vi "Upload_test_VI.vi"(8 "error in":errorcluster, 11 "SHz_selection":enum16{"10k", "100k"}(ring)) -> (0 "error out":errorcluster, 2 "selected F_array_Link":path[](array[path]), 3 "selected folder_List":string[](array[string]))   [LabVIEW 2018]
panel:
  in  "Add All Sample":bool
  in  "Add All":bool
  out "FOL#":i32
  out "x-1":u32
  out "SIDE":i32
  in  "Scrollbar V":i32(c297)
  out "Selected EX#":i32
  out "element":string
  in  "END":bool
  in  "All_Clear":bool
  in  "EX_IDX":i32
  out "Height":u32
  out "Top":i32
  out "Vertical":i32
  in  "selection":u16(ring) items=["backup (Rackstation)", "BR", "cadet", "COVID19", "Gynecologic Cancer", "HU", "KATO", "KATO2", "KATO3", "komoto", "Konno", "Kumamoto", "Kumamoto_N", "Lee", "Lee2", "Lee3", "LG_EX", "Lipid", "Numata_CHR", "Numata_MF", "Numata_N", "oligopeptide", "Pan_Cancer_N2", "Phi174", "Ryu", "Smoking"]
  out "1folder names":string[](array[string])
  out "Folder_List":string[](array[string])
  out "F_array_Link":path[](array[path])
  out "1st":path[](array[path])
  out "2nd":path[](array[path])
  out "logical OR 2":bool
  out "logical OR":bool
  out "foldername":string[](array[string])
  out "path":path
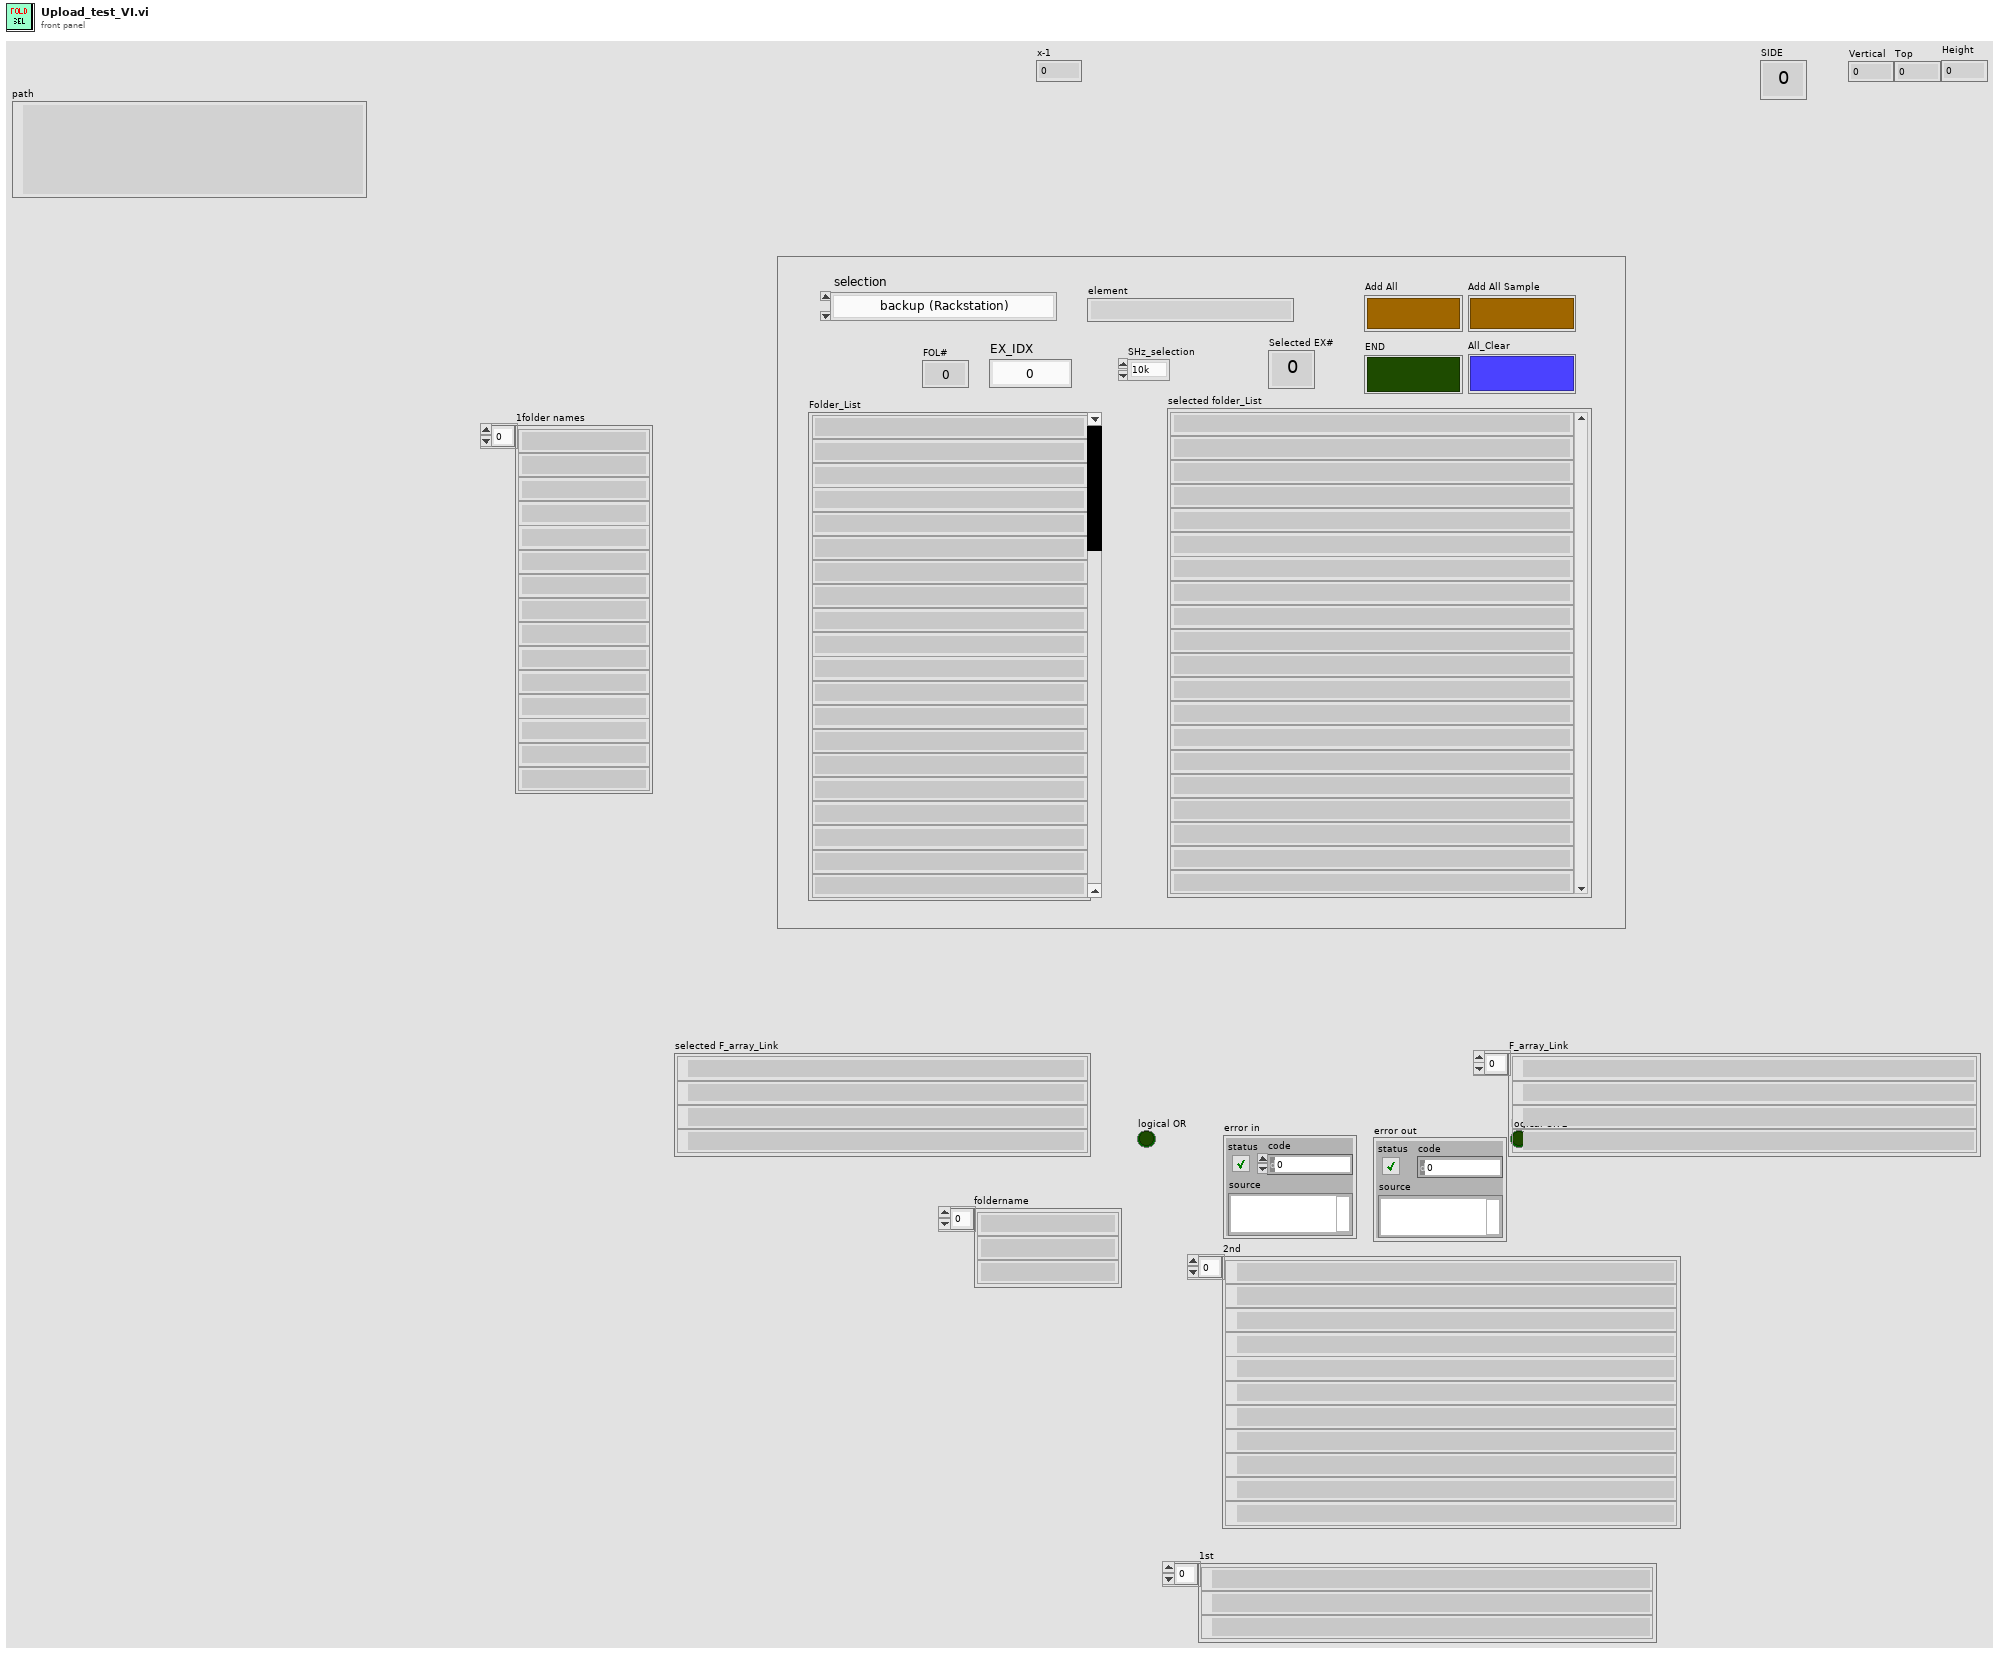
[diagram p1: front panel]
types:
  T1 = typedef "LVPoint32TypeDef.ctl" = cluster{"Horizontal":i32, "Vertical":i32}
  T2 = typedef "LVPositionTypeDef.ctl" = cluster{"Left":i32, "Top":i32}
  T3 = typedef "LVBoundsTypeDef.ctl" = cluster{"Width":u32, "Height":u32}
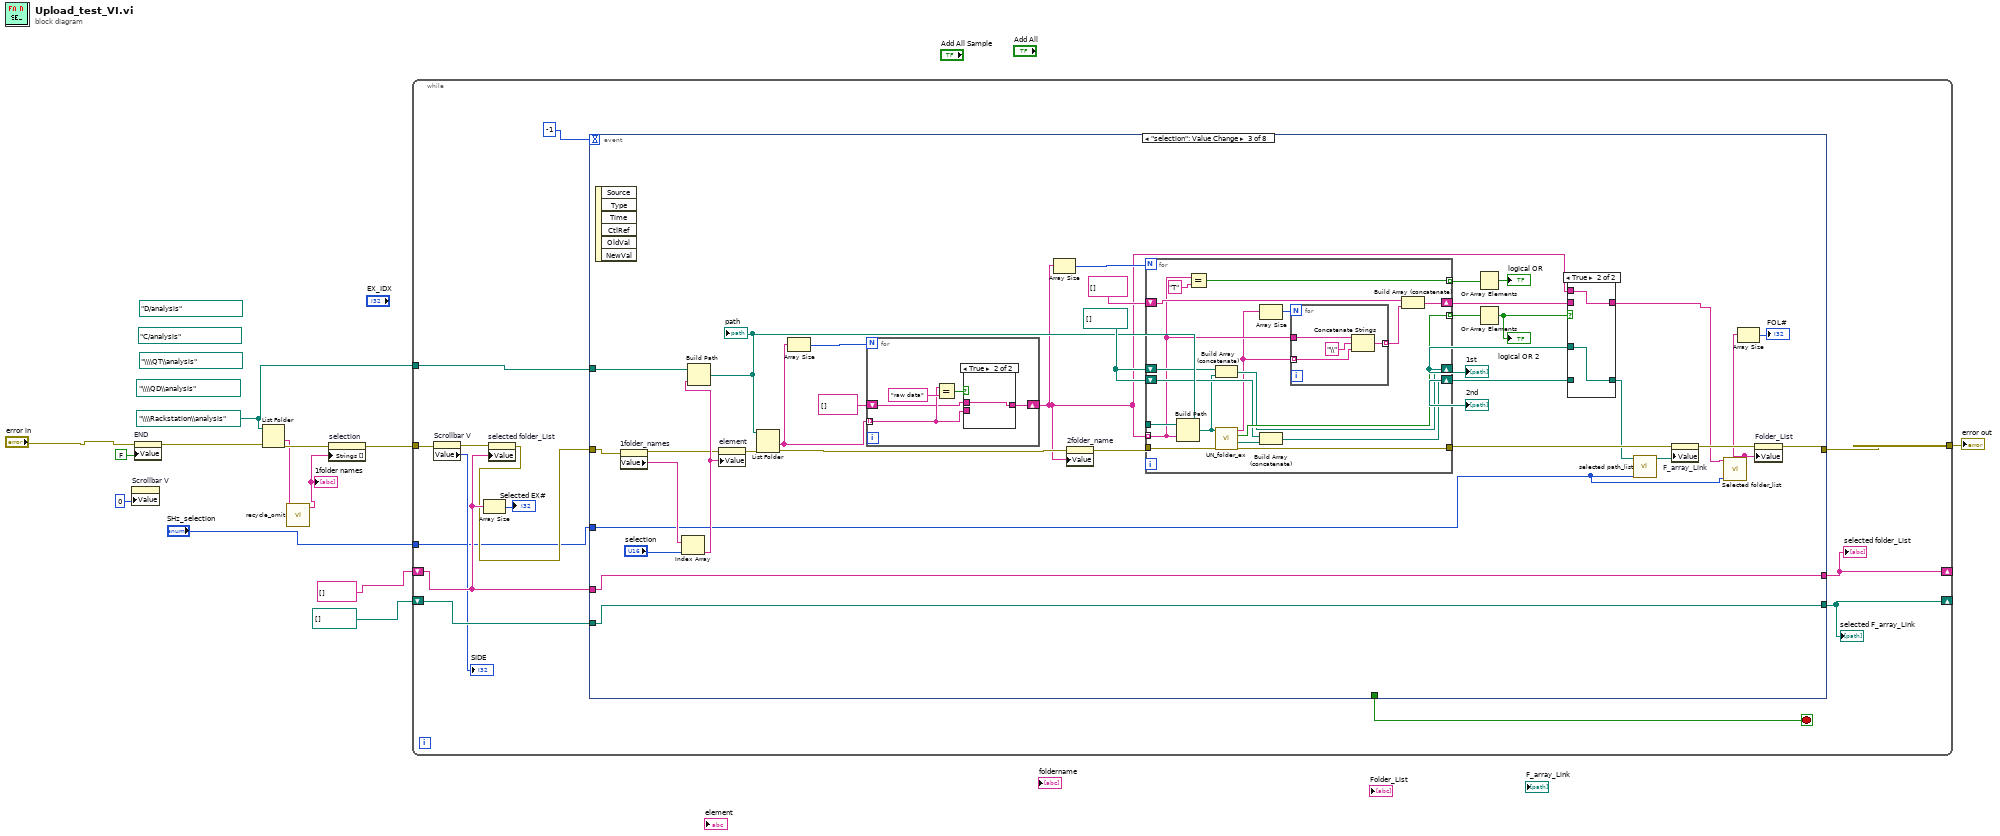
[diagram p0: block diagram]
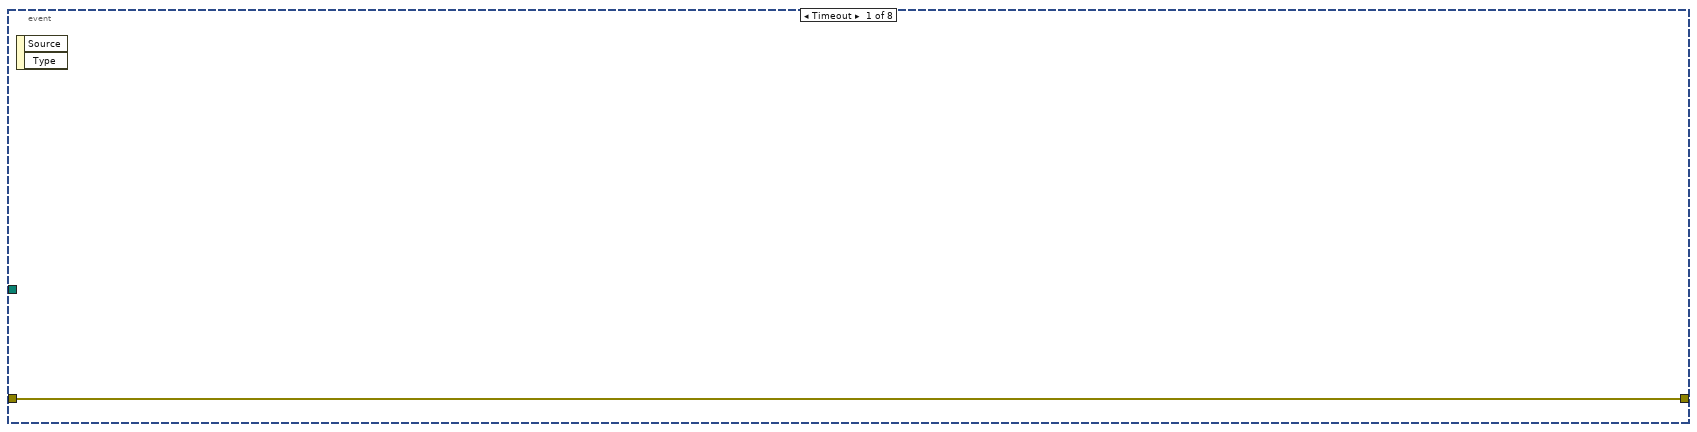
[diagram p2: hidden frame]
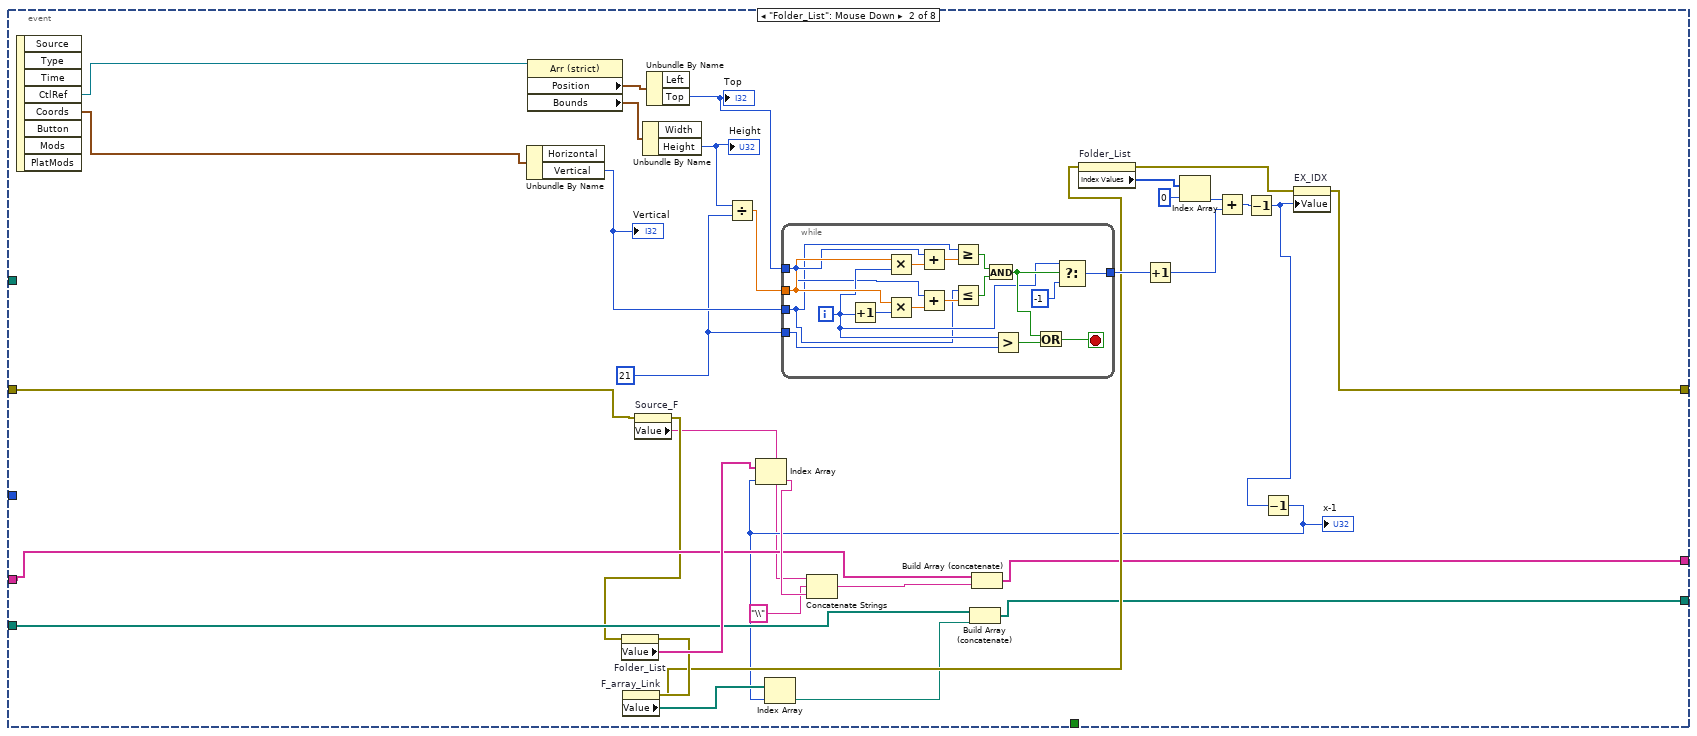
[diagram p3: hidden frame]
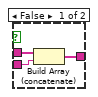
[diagram p5: hidden frame]
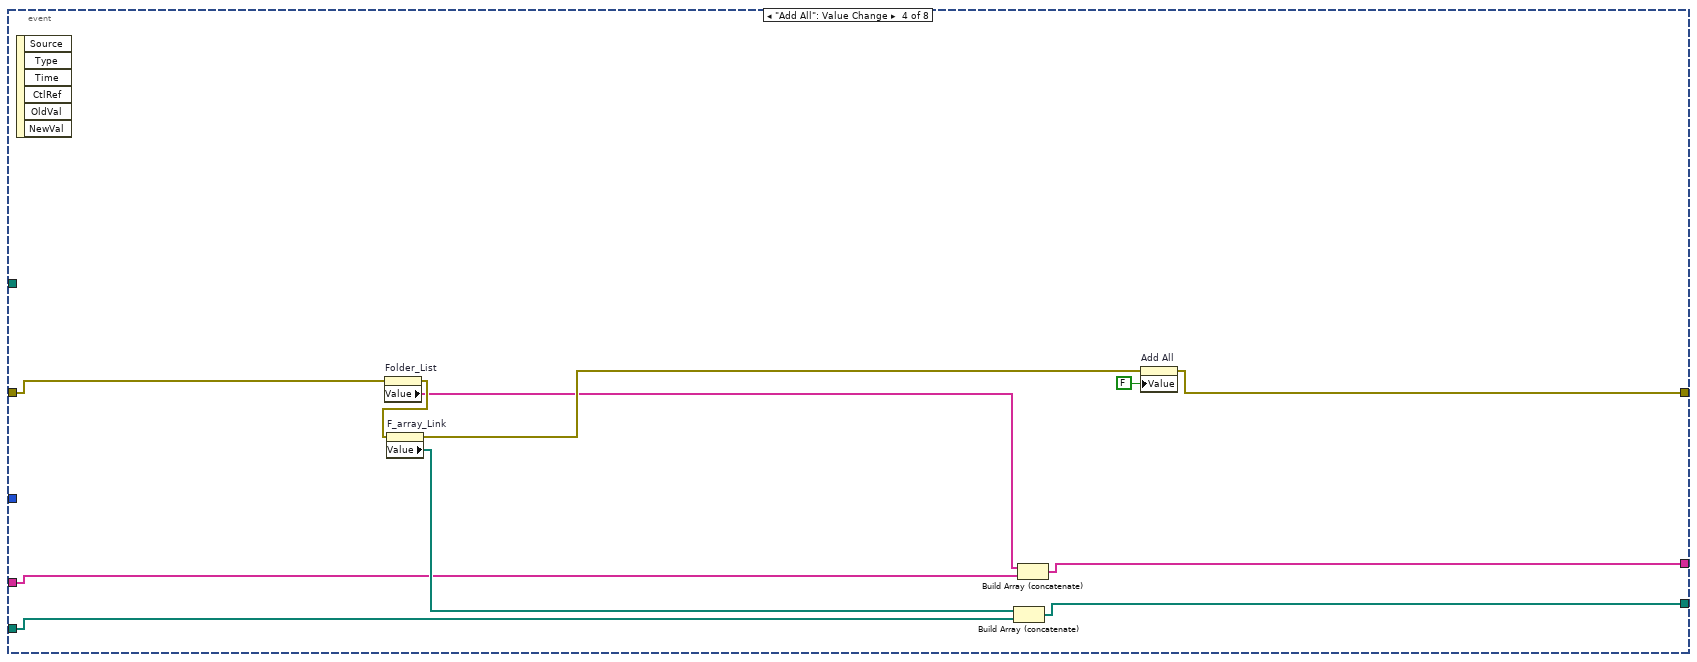
[diagram p6: hidden frame]
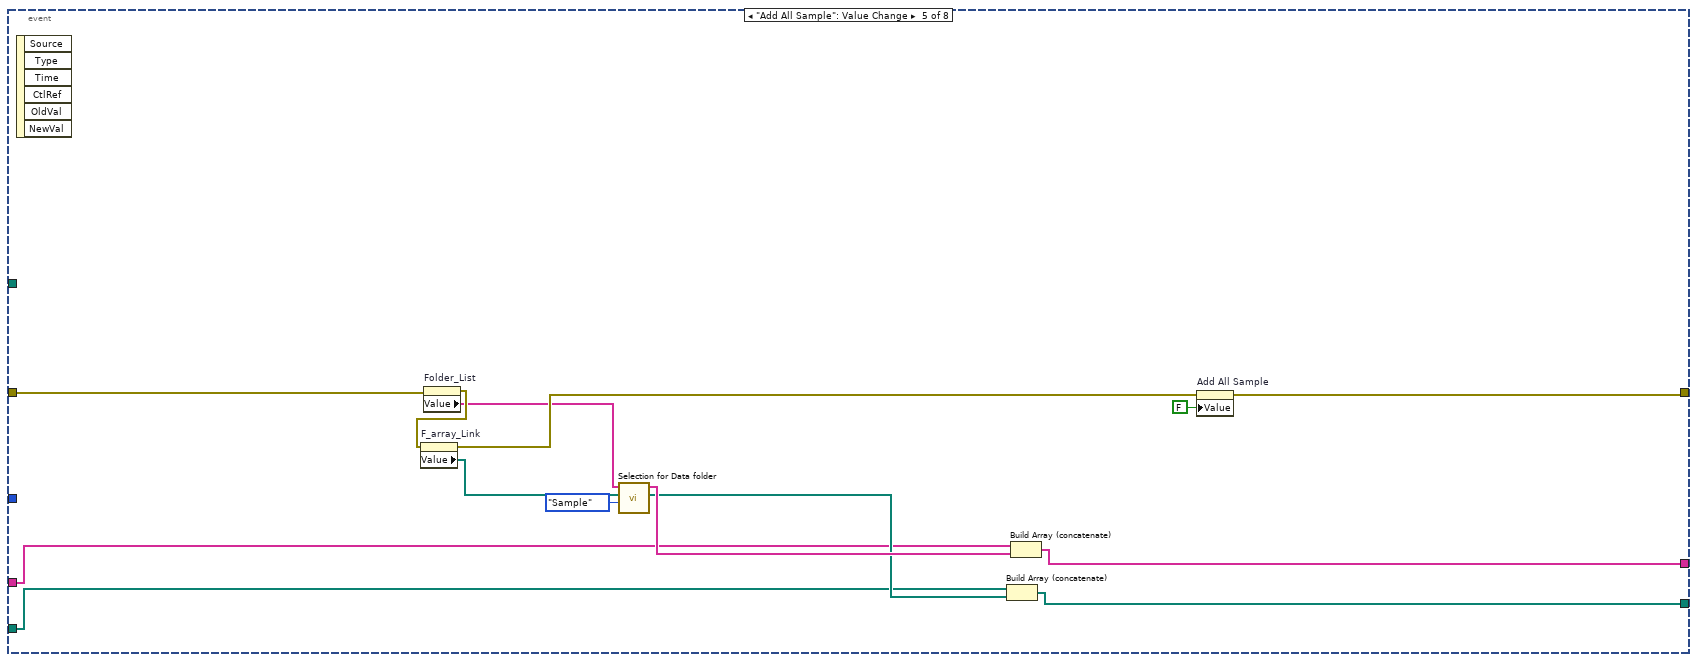
[diagram p7: hidden frame]
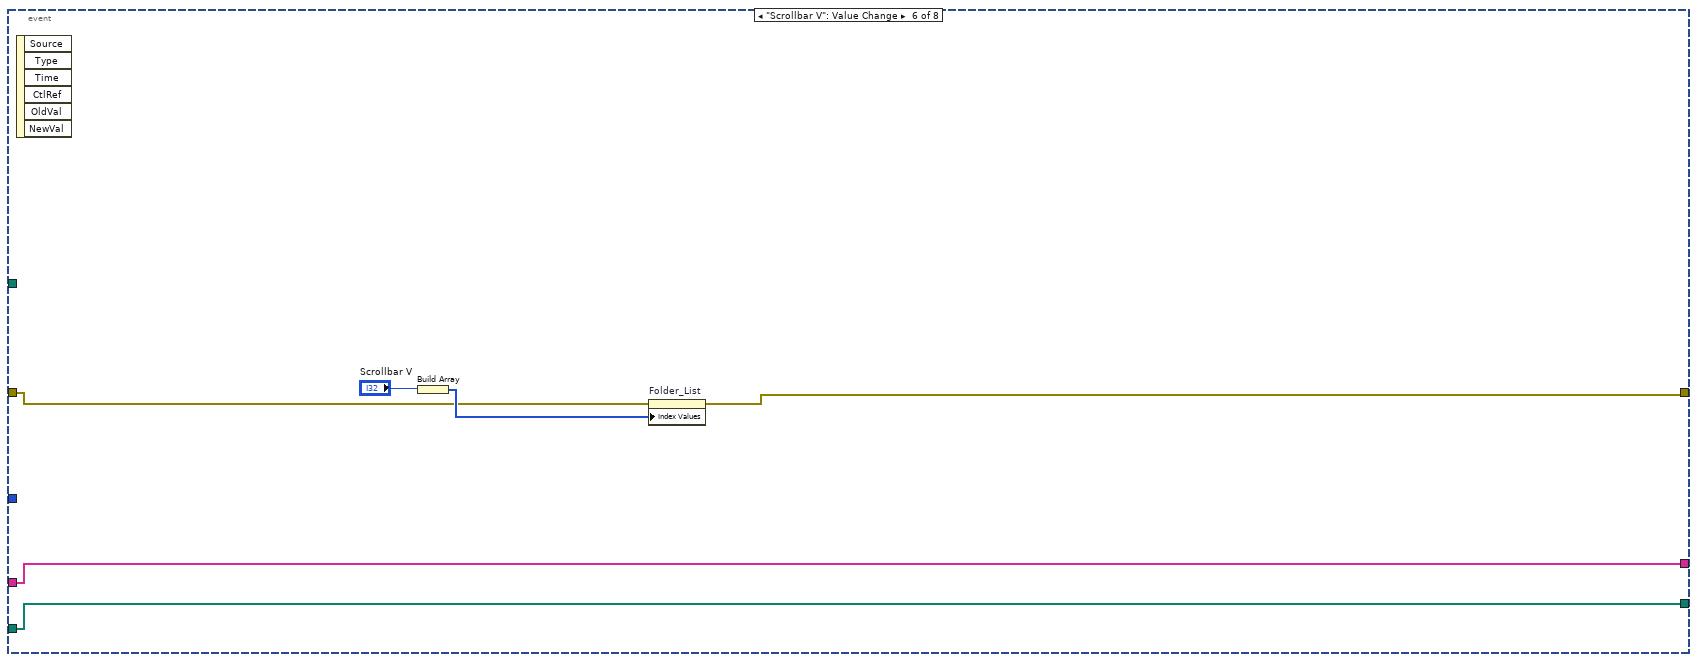
[diagram p8: hidden frame]
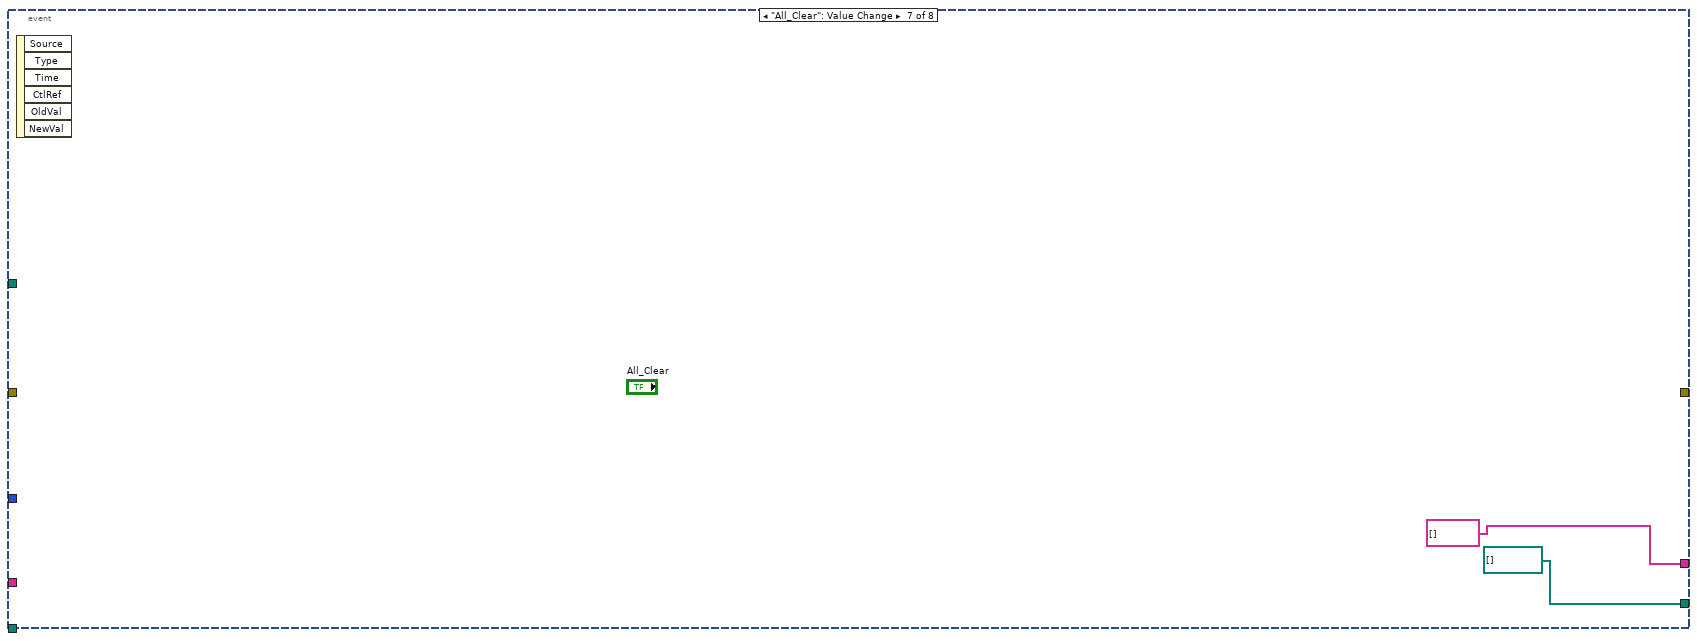
[diagram p9: hidden frame]
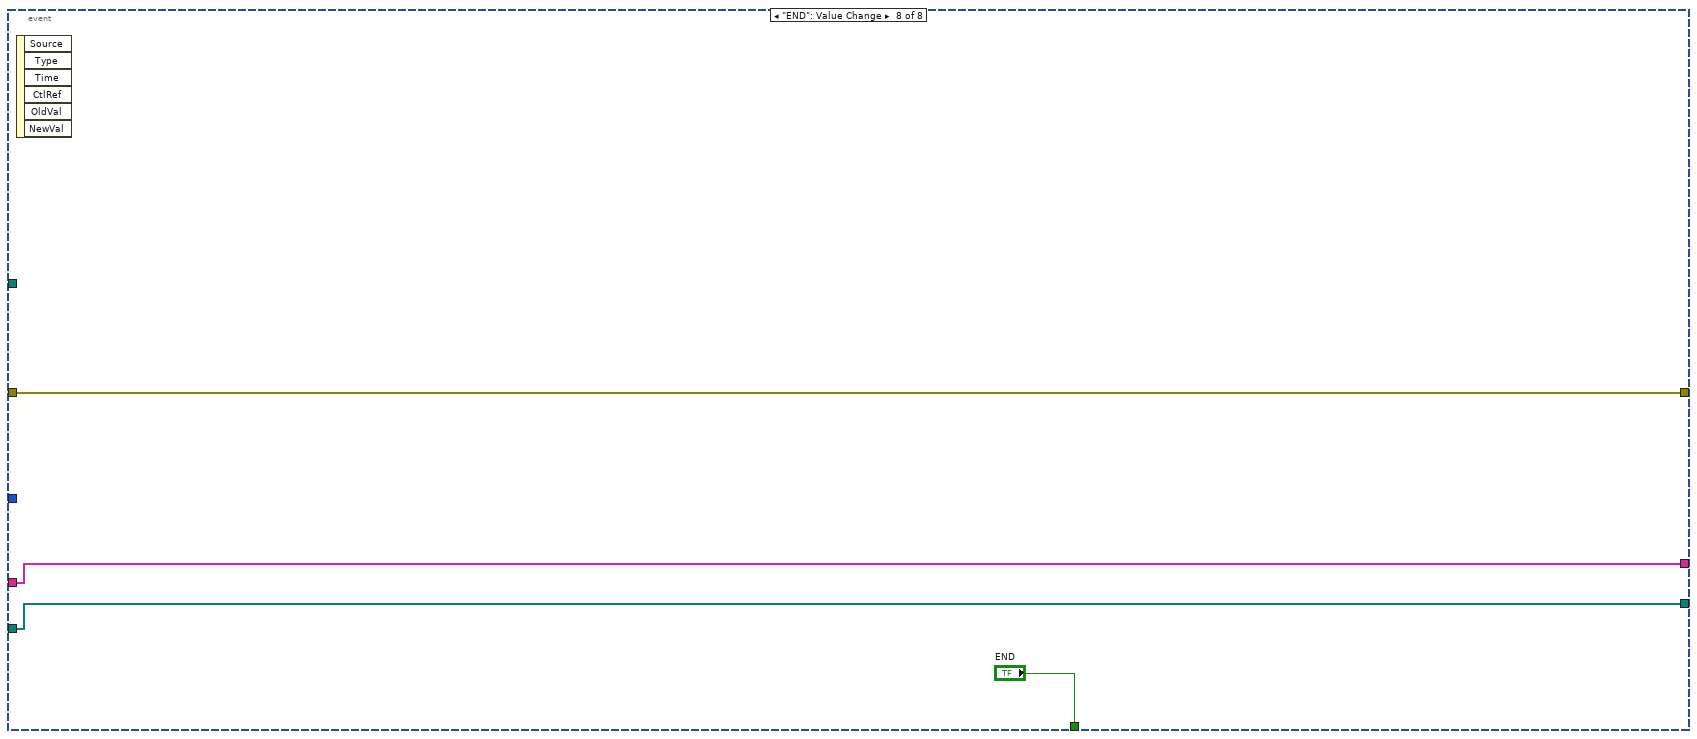
[diagram p10: hidden frame]
diagram:
  (unwired) path "D:/analysis"
  (unwired) path "C:/analysis"
  (unwired) path "\\\\QT\\analysis"
  (unwired) path "\\\\QD\\analysis"
  w10 = path "\\\\Rackstation\\analysis"
  n1 = property on="Scrollbar V" class="Scroll (strict)"("Value"=0 ("Scrollbar V")) -> ()  [unwired: 2 in, 2 out]
  n2 = property on="END" class="Bool (strict)"(error in="error in", "Value"=FALSE ("END")) -> (error out=w6:errorcluster)  [unwired: 1 in, 1 out]
  n3 = List Folder(path=w10, error in=w6) -> (folder names=w5:string[], error out=w13:errorcluster)  [unwired: 2 in, 2 out]
  n4 = call "recycle_omit.vi"("1folder names"=w5) -> ("Array"=w3:string[])  [unwired: 10 in]
  "1folder names" <- w3
  n5 = property on="selection" class="Ring (strict)"(error in=w13, "Strings []"=w3) -> (error out=w12:errorcluster)  [unwired: 1 in, 1 out]
  n6 = while {
    tunnel: w12 -> [w19]
    tunnel: [w27] -> w11
    tunnel: w10 -> [w25]
    shift-right: [w16] -> _
    shift-left: string[] [] -> [w21]
    shift-right: [w22] -> _
    shift-left: path[] [] -> [w23]
    tunnel: "SHz_selection" -> [w14]
    stop <- w24 stop-if-true
    n7 = property on="Scrollbar V" class="Scroll (strict)"(error in=w19) -> (error out=w18:errorcluster, "Value"=→"SIDE":i32)  [unwired: 1 in, 1 out]
    n8 = Array Size(array=w21) -> (size(s)=→"Selected EX#":i32)
    n9 = property on="selected folder_List" class="Arr (strict)"(error in=w18, "Value"=w21) -> (error out=w15:errorcluster)  [unwired: 1 in, 1 out]
    n10 = event shown="[2] \"selection\": Value Change" {
      selector: _ -> [_ _ _ _ _ _ _ _]
      dyn-events: _ -> [_ _ _ _ _ _ _ _]
      timeout: -1 -> [_ _ _ _ _ _ _ _]
      tunnel: w15 -> [w28 w32 w100 w160 w173 w179 _ w183]
      tunnel: [w28 w34 w91 w156 w170 w178 _ w183] -> w27
      tunnel: w25 -> [_ _ w98 _ _ _ _ _]
      tunnel: w21 -> [_ w37 w90 w150 w161 w176 _ w185]
      tunnel: [_ w36 w90 w154 w164 w176 string[] [] w185] -> w16
      tunnel: [_ _ _ _ _ _ _ "END"] -> w24
      tunnel: w23 -> [_ w38 w89 w151 w162 w175 _ w184]
      tunnel: [_ w35 w89 w153 w163 w175 path[] [] w184] -> w22
      tunnel: w14 -> [_ _ w83 _ _ _ _ _]
      event Timeout {
        n11 = event-data() -> ()  [unwired: 1 in, 2 out]
      }
      event "Folder_List": Mouse Down {
        w42 = 21 ("f")
        n12 = event-data() -> ("CtlRef"=w39:refnum<vi>, "Coords"=w40:T1)  [unwired: 1 in, 6 out]
        n13 = Unbundle By Name(w40) -> ("Vertical"=w59:i32)  [unwired: 1 out]
        "Vertical" <- w59
        n14 = property class="Arr (strict)"(reference=w39) -> ("Position"=w61:T2, "Bounds"=w60:T3)  [unwired: 1 in, 2 out]
        n15 = property on="Source_F" class="Str"(error in=w32) -> (error out=w31:errorcluster, "Value"=w30:string)  [unwired: 1 in, 1 out]
        n16 = property on="Folder_List" class="Arr (strict)"(error in=w31) -> (error out=w47:errorcluster, "Value"=w51:string[])  [unwired: 1 in, 1 out]
        n17 = property on="F_array_Link" class="Arr (strict)"(error in=w47) -> (error out=w46:errorcluster, "Value"=w45:path[])  [unwired: 1 in, 1 out]
        n18 = Unbundle By Name(w60) -> ("Height"=w58:u32)  [unwired: 1 out]
        "Height" <- w58
        n19 = Unbundle By Name(w61) -> ("Top"=w56:i32)  [unwired: 1 out]
        "Top" <- w56
        n20 = Divide(x=w58, y=w42) -> (x/y=w57:dbl)
        n21 = while {
          tunnel: w59 -> [w63]
          tunnel: w57 -> [w69]
          tunnel: w56 -> [w65]
          tunnel: [w74] -> w52
          tunnel: w42 -> [w64]
          i -> [w68]
          stop <- w72 stop-if-true
          n22 = Increment(x=w68) -> (x+1=w79:i32)
          n23 = Multiply(x=w69, y=w68) -> (x*y=w66:dbl)
          n24 = Multiply(x=w69, y=w79) -> (x*y=w77:dbl)
          n25 = Add(x=w65, y=w66) -> (x+y=w67:dbl)
          n26 = Add(x=w65, y=w77) -> (x+y=w78:dbl)
          n27 = Greater Or Equal?(x=w63, y=w67) -> (x >= y?=w76:bool)
          n28 = Less Or Equal?(x=w63, y=w78) -> (x <= y?=w75:bool)
          n29 = And(x=w76, y=w75) -> (x .and. y?=w71:bool)
          n30 = Greater?(x=w68, y=w64) -> (0:w70:bool)
          n31 = Or(x=w71, y=w70) -> (x .or. y?=w72:bool)
          n32 = Select(t=w68, s=w71, f=-1) -> (s? t:f=w74:i32)
        }
        n33 = property on="Folder_List" class="Arr (strict)"(error in=w46) -> (error out=w49:errorcluster, "Index Values"=w62:u32[])  [unwired: 1 in, 1 out]
        n34 = Increment(x=w52) -> (x+1=w55:i32)
        n35 = Index Array(array=w62, index=0 ("指標")) -> (element=w53:u32)
        n36 = Add(x=w53, y=w55) -> (x+y=w54:u32)
        n37 = Decrement(x=w54) -> (x-1=w29:u32)
        n38 = Decrement(x=w29) -> (x-1=w33:u32)
        "x-1" <- w33
        n39 = Index Array(array=w51, index=w33) -> (element=w50:string)
        n40 = Index Array(array=w45, index=w33) -> (element=w44:path)
        n41 = Concatenate Strings(w30, "\\" ("string"), w50) -> (w48:string)
        n42 = Build Array (concatenate)(w38, w44) -> (w35:path[])
        n43 = Build Array (concatenate)(w37, w48) -> (w36:string[])
        n44 = property on="EX_IDX" class="DigNum (strict)"(error in=w49, "Value"=w29) -> (error out=w34:errorcluster)  [unwired: 1 in, 1 out]
      }
      event "selection": Value Change {
        w103 = path[] []
        n45 = event-data() -> ()  [unwired: 1 in, 6 out]
        n46 = property on="1folder_names" class="Arr (strict)"(error in=w100) -> (error out=w87:errorcluster, "Value"=w99:string[])  [unwired: 1 in, 1 out]
        n47 = Index Array(array=w99, index="selection") -> (element=w88:string)
        n48 = Build Path(base path=w98, name or relative path=w88) -> (appended path=w97:path)
        "path" <- w97
        n49 = property on="element" class="Str"(error in=w87, "Value"=w88) -> (error out=w86:errorcluster)  [unwired: 1 in, 1 out]
        n50 = List Folder(path=w97, error in=w86) -> (folder names=w109:string[], error out=w96:errorcluster)  [unwired: 2 in, 2 out]
        n51 = Array Size(array=w109) -> (size(s)=w110:i32)
        n52 = for {
          N: w110 -> [_]
          tunnel: w109 -> [w121] mode=indexing
          shift-right: [w120] -> w95
          shift-left: string[] [] -> [w119]
          n53 = Equal?(x=w121, y="raw data") -> (x = y?=w122:bool)
          n54 = case shown="True" w122 {
            tunnel: w121 -> [w126 _]
            tunnel: [w125 w127] -> w120
            tunnel: w119 -> [w124 w127]
            frame False {
              n55 = Build Array (concatenate)(w124, w126) -> (w125:string[])
            }
            frame True {
            }
          }
        }
        n56 = Array Size(array=w95) -> (size(s)=w114:i32)
        n57 = property on="2folder_name" class="Arr (strict)"(error in=w96, "Value"=w95) -> (error out=w94:errorcluster)  [unwired: 1 in, 1 out]
        n58 = for {
          N: w114 -> [_]
          tunnel: w95 -> [w130] mode=indexing
          tunnel: w94 -> [w142]
          tunnel: [w144] -> w113 mode=indexing
          tunnel: w97 -> [w143]
          tunnel: [w141] -> w93
          tunnel: [w140] -> w111 mode=indexing
          shift-right: [w138] -> w107
          shift-left: w103 -> [w137]
          shift-right: [w135] -> w106
          shift-left: w103 -> [w134]
          shift-right: [w133] -> w105
          shift-left: string[] [] -> [w132]
          n59 = Build Path(base path=w143, name or relative path=w130) -> (appended path=w136:path)
          n60 = Equal?(x=w130, y="T" ("regular expression")) -> (x = y?=w144:bool)
          n61 = Build Array (concatenate)(w134, w136) -> (w135:path[])
          n62 = call "UN_folder_ex.vi"("error in"=w142, "path"=w136) -> ("error out"=w141:errorcluster, "Array"=w139:path[], "logical OR"=w140:bool, "foldername"=w129:string[])  [unwired: 6 in]
          n63 = Array Size(array=w129) -> (size(s)=w131:i32)
          n64 = Build Array (concatenate)(w137, w139) -> (w138:path[])
          n65 = for {
            N: w131 -> [_]
            tunnel: w130 -> [w149]
            tunnel: w129 -> [w148] mode=indexing
            tunnel: [w146] -> w128 mode=indexing
            n66 = Concatenate Strings(w149, "\\" ("string"), w148) -> (w146:string)
          }
          n67 = Build Array (concatenate)(w132, w128) -> (w133:string[])
        }
        "2nd" <- w107
        "1st" <- w106
        n68 = Or Array Elements(Boolean array=w113) -> (logical OR=→"logical OR":bool)
        n69 = Or Array Elements(Boolean array=w111) -> (logical OR=w108:bool)
        "logical OR 2" <- w108
        n70 = case shown="True" w108 {
          tunnel: w107 -> [w116 _]
          tunnel: [w116 w118] -> w85
          tunnel: w106 -> [_ w118]
          tunnel: w95 -> [_ w117]
          tunnel: w105 -> [w115 _]
          tunnel: [w115 w117] -> w82
          frame False {
          }
          frame True {
          }
        }
        n71 = call "selected path_list.vi"("selection"=w83, "F_array_Link"=w85) -> ("Selected F_array_Link"=w84:path[])  [unwired: 9 in]
        n72 = property on="F_array_Link" class="Arr (strict)"(error in=w93, "Value"=w84) -> (error out=w92:errorcluster)  [unwired: 1 in, 1 out]
        n73 = call "Selected folder_list.vi"("selection"=w83, "Folder_List"=w82) -> ("selected Folder List"=w80:string[])  [unwired: 9 in]
        n74 = Array Size(array=w80) -> (size(s)=→"FOL#":i32)
        n75 = property on="Folder_List" class="Arr (strict)"(error in=w92, "Value"=w80) -> (error out=w91:errorcluster)  [unwired: 1 in, 1 out]
      }
      event "Add All": Value Change {
        n76 = event-data() -> ()  [unwired: 1 in, 6 out]
        n77 = property on="Folder_List" class="Arr (strict)"(error in=w160) -> (error out=w159:errorcluster, "Value"=w155:string[])  [unwired: 1 in, 1 out]
        n78 = property on="F_array_Link" class="Arr (strict)"(error in=w159) -> (error out=w158:errorcluster, "Value"=w152:path[])  [unwired: 1 in, 1 out]
        n79 = Build Array (concatenate)(w152, w151) -> (w153:path[])
        n80 = Build Array (concatenate)(w155, w150) -> (w154:string[])
        n81 = property on="Add All" class="Bool (strict)"(error in=w158, "Value"=FALSE ("Add All")) -> (error out=w156:errorcluster)  [unwired: 1 in, 1 out]
      }
      event "Add All Sample": Value Change {
        n82 = event-data() -> ()  [unwired: 1 in, 6 out]
        n83 = property on="Folder_List" class="Arr (strict)"(error in=w173) -> (error out=w172:errorcluster, "Value"=w169:string[])  [unwired: 1 in, 1 out]
        n84 = property on="F_array_Link" class="Arr (strict)"(error in=w172) -> (error out=w171:errorcluster, "Value"=w168:path[])  [unwired: 1 in, 1 out]
        n85 = call "Selection for Data folder.vi"("Select"=enum16{"Sample", "Blank"}."Sample", "F_array_Link"=w168, "Folder_List"=w169) -> ("S_F_array_Link"=w165:path[], "S_Folder_List"=w166:string[])  [unwired: 7 in]
        n86 = Build Array (concatenate)(w162, w165) -> (w163:path[])
        n87 = Build Array (concatenate)(w161, w166) -> (w164:string[])
        n88 = property on="Add All Sample" class="Bool (strict)"(error in=w171, "Value"=FALSE ("Add All Sample")) -> (error out=w170:errorcluster)  [unwired: 1 in, 1 out]
      }
      event "Scrollbar V": Value Change {
        n89 = event-data() -> ()  [unwired: 1 in, 6 out]
        n90 = Build Array("Scrollbar V") -> (w180:i32[])
        n91 = property on="Folder_List" class="Arr (strict)"(error in=w179, "Index Values"=w180) -> (error out=w178:errorcluster)  [unwired: 1 in, 1 out]
      }
      event "All_Clear": Value Change {
        n92 = event-data() -> ()  [unwired: 1 in, 6 out]
      }
      event "END": Value Change {
        n93 = event-data() -> ()  [unwired: 1 in, 6 out]
      }
    }
    "selected F_array_Link" <- w22
    "selected folder_List" <- w16
  }
  "error out" <- w11
